vi "Tool_Unicode Update Table Headers.vi"(7 "Interpret as Unicode (T)":bool=TRUE, 8 "error in (no error)":errorcluster, 9 "Row Headers[]":string[](array[string]), 10 "Column Headers[]":string[](array[string]), 11 "Table Ref":refnum<vi>) -> (0 "error out":errorcluster, 3 "Table Ref":refnum<vi>)   [LabVIEW 2019, in "Language Selection.lvlib"]
doc: "Uses \"Column Headers[]\" and \"Row Headers[]\" input arrays to translate Table headers.\n- - -\nCopyright (c) 2026, Merecs Engineering GmbH"
uses:
  Language Selection.lvlib
panel:
  # "Connector Pane"
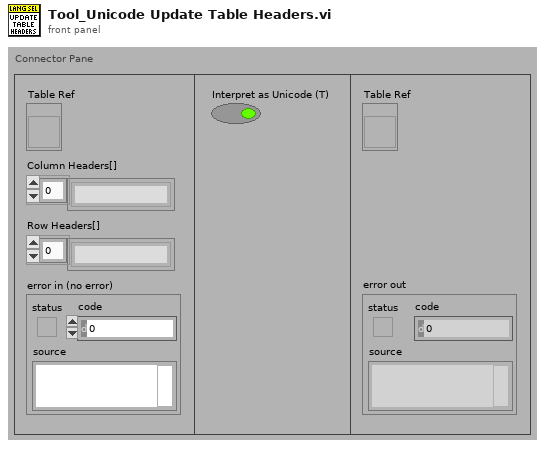
[diagram p1: front panel]
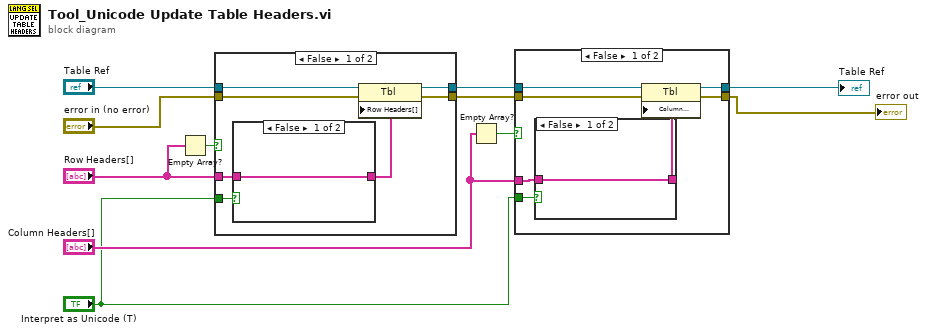
[diagram p0: block diagram]
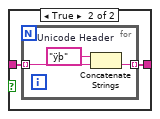
[diagram p2: hidden frame]
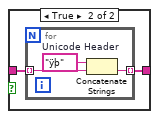
[diagram p4: hidden frame]
diagram:
  n1 = Empty Array?(array="Row Headers[]") -> (empty?=w8:bool)
  n2 = case shown="False" w8 {
    tunnel: "Row Headers[]" -> [w18 _]
    tunnel: "Table Ref" -> [w16 w26]
    tunnel: "error in (no error)" -> [w15 w25]
    tunnel: [w14 w26] -> w9
    tunnel: "Interpret as Unicode (T)" -> [w13 _]
    tunnel: [w12 w25] -> w4
    frame False {
      n3 = case shown="False" w13 {
        tunnel: w18 -> [w19 w21]
        tunnel: [w19 w20] -> w17
        frame False {
        }
        frame True {
          n4 = for {
            tunnel: w21 -> [w24] mode=indexing
            tunnel: [w23] -> w20 mode=indexing
            w22 = "ÿþ"  # Unicode Header
            n5 = Concatenate Strings(w22, w24) -> (w23:string)
          }
        }
      }
      n6 = property class="Tbl"(reference=w16, error in=w15, "Row Headers[]"=w17) -> (reference out=w14:refnum<vi>, error out=w12:errorcluster)
    }
    frame True {
    }
  }
  n7 = Empty Array?(array="Column Headers[]") -> (empty?=w5:bool)
  n8 = case shown="False" w5 {
    tunnel: "Column Headers[]" -> [w33 _]
    tunnel: [w32 w41] -> w3
    tunnel: w4 -> [w30 w41]
    tunnel: w9 -> [w29 w40]
    tunnel: "Interpret as Unicode (T)" -> [w28 _]
    tunnel: [w27 w40] -> w2
    frame False {
      n9 = case shown="False" w28 {
        tunnel: w33 -> [w34 w36]
        tunnel: [w34 w35] -> w31
        frame False {
        }
        frame True {
          n10 = for {
            tunnel: w36 -> [w39] mode=indexing
            tunnel: [w38] -> w35 mode=indexing
            w37 = "ÿþ"  # Unicode Header
            n11 = Concatenate Strings(w37, w39) -> (w38:string)
          }
        }
      }
      n12 = property class="Tbl"(reference=w29, error in=w30, "Column Headers[]"=w31) -> (reference out=w27:refnum<vi>, error out=w32:errorcluster)
    }
    frame True {
    }
  }
  "error out" <- w3
  "Table Ref" <- w2
